vi "NLTest_exit.vi"(8 "error in (no error)":errorcluster, 11 "NLTest in":refnum<class "NLTest.lvclass">) -> (0 "error out":errorcluster)   [LabVIEW 2017, in "NLTest.lvclass"]
uses:
  NLTest.lvclass
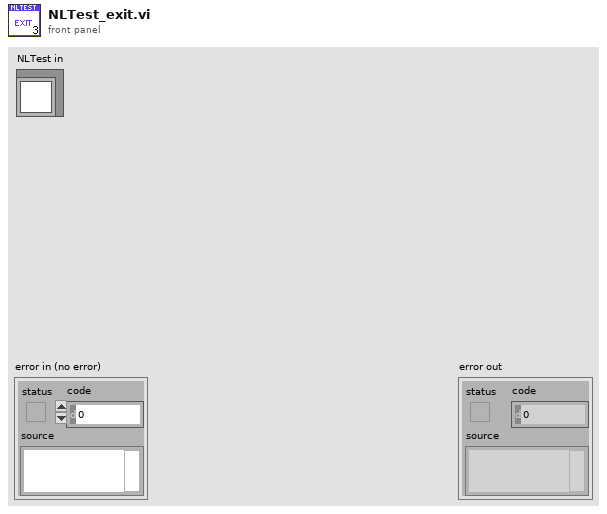
[diagram p1: front panel]
types:
  T1 = enum32{"Invalid", "Standard", "Closed", "Hidden", "Minimized", "Maximized"}
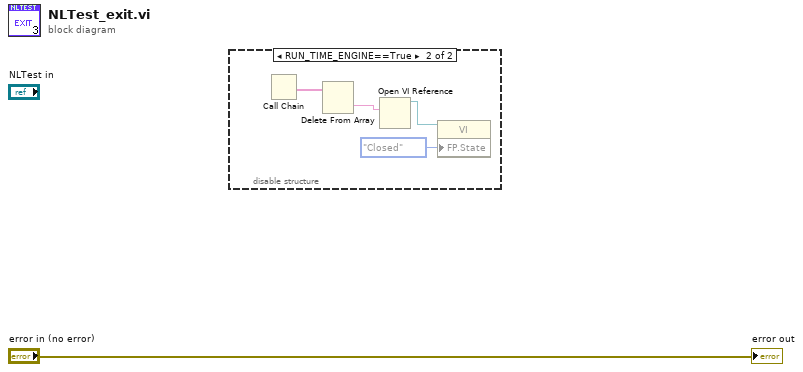
[diagram p0: block diagram]
diagram:
  n1 = disable-structure shown="RUN_TIME_ENGINE==True" {
    frame condition #0 (active) {
    }
    frame condition #1 {
      n2 = Call Chain() -> (call chain=w4:string[])
      n3 = Delete From Array(array=w4) -> (deleted portion=w3:string)  [unwired: 2 in, 1 out]
      n4 = Open VI Reference(vi path=w3) -> (vi reference=w2:refnum<vi>)  [unwired: 5 in, 1 out]
      n5 = property class="VI"(reference=w2, "FP.State"=T1."Closed" ("前面板窗口:状态")) -> ()  [unwired: 1 in, 2 out]
    }
  }
  "error out" <- "error in (no error)"
